vi "File Size Rollover_Log Record Exceeds Threshold.vi"() -> ()   [LabVIEW 2018]
uses:
  src/api/logger_class/Log Levels.ctl
  src/api/configuration/formatters/format_string_formatter/Format String.lvclass
  C:/Users/Colin/Documents/software_projects/labview/glog/src/api/extension/formatter_interface/Formatter.lvclass
  src/api/configuration/handlers/file_handler/File Handler.lvclass
  C:/Users/Colin/Documents/software_projects/labview/glog/src/api/extension/formatting_handler_interface/Formatting Handler.lvclass
  src/api/logger_class/Log (Parts).vi
  src/api/logger_class/Logger.lvclass
panel:
  out "3 files?":bool caption="1 file? (1st)"
  out "2 files?":bool caption="1 file? (1st)"
  in  "delete when done?":bool=TRUE
  out "error out":errorcluster
  out "1 file?":bool caption="1 file? (1st)"
  # "Locals"
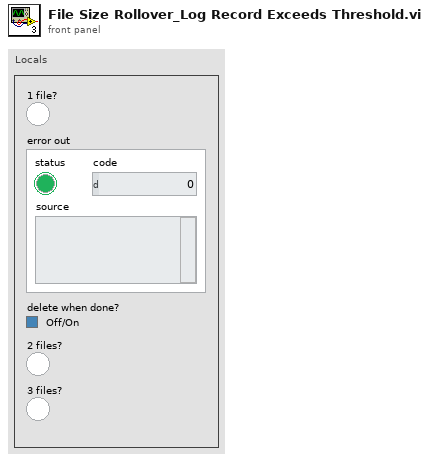
[diagram p1: front panel]
types:
  T1 = typedef "GLog.lvlib/Logger.lvclass/Log Levels.ctl" = enum16{"Trace", "Debug", "Info", "Warning", "Error", "Critical"}
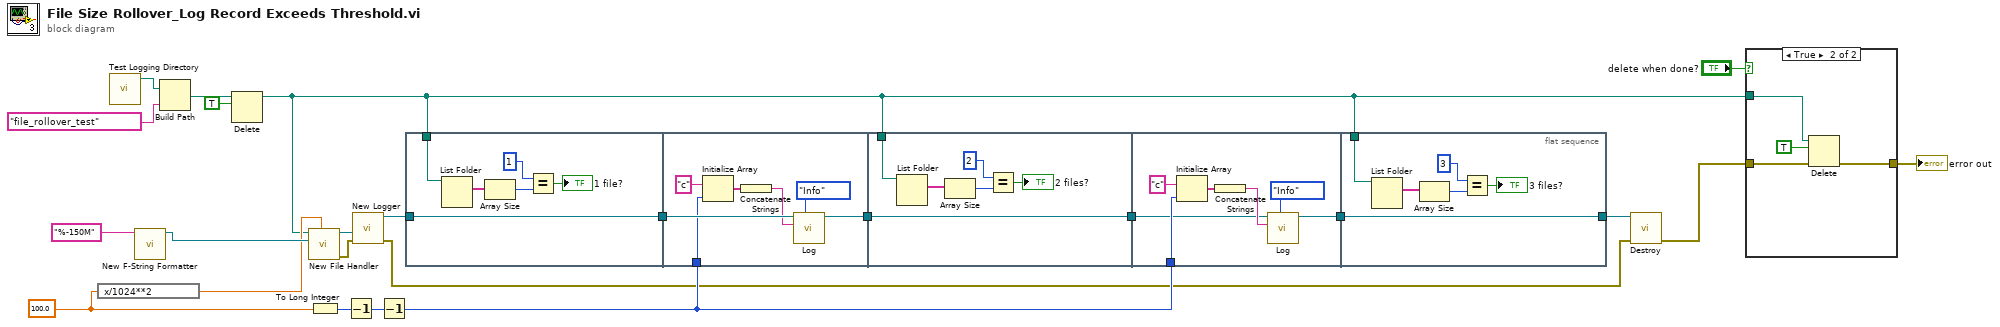
[diagram p0: block diagram]
diagram:
  w17 = 100.0
  n1 = expression code="x/1024**2"(w17) -> (w4:dbl)
  n2 = call "Test Logging Directory.vi"() -> ("test logging directory"=w7:path)  [unwired: 11 in]
  n3 = call "New F-String Formatter.vi"("format string (\"%T | %L | %M\")"="%-150M" ("format string (\"%T | %L | %M\")")) -> ("new f-string formatter"=w16:refnum<class "Format String.lvclass">)  [unwired: 10 in]
  n4 = Build Path(base path=w7, name or relative path="file_rollover_test") -> (appended path=w2:path)
  n5 = Delete(path (use dialog)=w2, entire hierarchy (F)=TRUE) -> (deleted path=w1:path)  [unwired: 3 in, 2 out]
  n6 = call "New File Handler.vi"("max file size [MB](50)"=w4, "formatter (JSON)"=w16, "log directory (<app dir>/logs)"=w1) -> ("error out"=w5:errorcluster, "file handler"=w24:refnum<class "File Handler.lvclass">)  [unwired: 6 in, 1 out]
  n7 = To Long Integer(number=w17) -> (32bit integer=w13:i32)
  n8 = Decrement(x=w13) -> (x-1=w10:i32)
  n9 = call "New Logger.vi"("error in (no error)"=w5, "log handler (file handler)"=w24) -> ("error out"=w6:errorcluster, "logger"=w20:refnum<class "Logger.lvclass">)  [unwired: 8 in]
  n10 = Decrement(x=w10) -> (x-1=w9:i32)
  n11 = flat-sequence {
    tunnel: w20 -> [w30]
    tunnel: [w30] -> w19
    tunnel: w1 -> [w26]
    tunnel: [w35] -> w21
    tunnel: w19 -> [w36]
    tunnel: w9 -> [w31]
    tunnel: w1 -> [w43]
    tunnel: w21 -> [w42]
    tunnel: [w42] -> w14
    tunnel: w14 -> [w44]
    tunnel: w9 -> [w45]
    tunnel: [w46] -> w12
    tunnel: [w56] -> w11
    tunnel: w12 -> [w56]
    tunnel: w1 -> [w51]
    frame #0 {
      n12 = List Folder(path=w26) -> (filenames=w27:string[])  [unwired: 3 in, 3 out]
      n13 = Array Size(array=w27) -> (size(s)=w28:i32)
      n14 = Equal?(x=1, y=w28) -> (x = y?=→"1 file?":bool)
    }
    frame #1 {
      n15 = Initialize Array("c" ("message"), w31) -> (w33:string[])
      n16 = Concatenate Strings(w33) -> (w32:string)
      n17 = call-poly "Log.vi"("log level"=Log_Levels."Info" ("level"), "message"=w32, "logger in"=w36) -> ("logger out"=w35:refnum<class "Logger.lvclass">)  [unwired: 8 in]
    }
    frame #2 {
      n18 = List Folder(path=w43) -> (filenames=w38:string[])  [unwired: 3 in, 3 out]
      n19 = Array Size(array=w38) -> (size(s)=w40:i32)
      n20 = Equal?(x=2, y=w40) -> (x = y?=→"2 files?":bool)
    }
    frame #3 {
      n21 = Initialize Array("c" ("message"), w45) -> (w48:string[])
      n22 = Concatenate Strings(w48) -> (w47:string)
      n23 = call-poly "Log.vi"("log level"=Log_Levels."Info" ("level"), "message"=w47, "logger in"=w44) -> ("logger out"=w46:refnum<class "Logger.lvclass">)  [unwired: 8 in]
    }
    frame #4 {
      n24 = List Folder(path=w51) -> (filenames=w52:string[])  [unwired: 3 in, 3 out]
      n25 = Array Size(array=w52) -> (size(s)=w54:i32)
      n26 = Equal?(x=3, y=w54) -> (x = y?=→"3 files?":bool)
    }
  }
  n27 = call "Destroy.vi"("error in (no error)"=w6, "logger in"=w11) -> ("error out"=w8:errorcluster)  [unwired: 8 in, 1 out]
  n28 = case shown="True" "delete when done?" {
    tunnel: w1 -> [_ w59]
    tunnel: [_ w58] -> w23
    tunnel: w8 -> [_ w57]
    frame False {
    }
    frame True {
      n29 = Delete(path (use dialog)=w59, entire hierarchy (F)=TRUE, error in=w57) -> (error out=w58:errorcluster)  [unwired: 2 in, 2 out]
    }
  }
  "error out" <- w23
